vi "SetReadTrigger.vi"() -> ()   [LabVIEW 2015]
panel:
  out "触发状态":string
  in  "VISA资源名称":refnum<visa-resource-name>
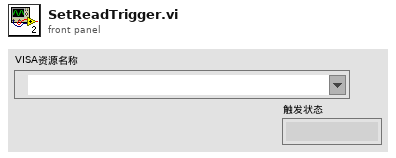
[diagram p1: front panel]
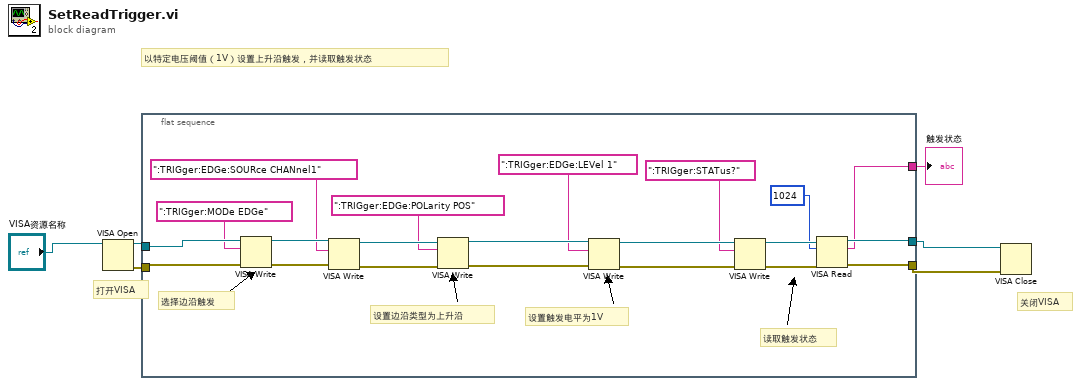
[diagram p0: block diagram]
diagram:
  # "关闭VISA"
  # "打开VISA"
  # "以特定电压阈值（1V）设置上升沿触发，并读取触发状态"
  n1 = VISA Open(VISA resource name="VISA资源名称") -> (VISA resource name=w6:refnum<visa-resource-name>, error out=w5:errorcluster)  [unwired: 4 in]
  n2 = flat-sequence {
    tunnel: w6 -> [w27]
    tunnel: w5 -> [w26]
    tunnel: [w11] -> w3
    tunnel: [w9] -> w2
    tunnel: [w7] -> w1
    frame #0 {
      # "设置触发电平为1V"
      # "设置边沿类型为上升沿"
      # "读取触发状态"
      # "选择边沿触发"
      n3 = VISA Write(VISA resource name=w27, write buffer=":TRIGger:MODe EDGe", error in (no error)=w26) -> (VISA resource name out=w24:refnum<visa-resource-name>, error out=w22:errorcluster)  [unwired: 1 out]
      n4 = VISA Write(VISA resource name=w24, write buffer=":TRIGger:EDGe:SOURce CHANnel1" ("写入缓冲区"), error in (no error)=w22) -> (VISA resource name out=w23:refnum<visa-resource-name>, error out=w21:errorcluster)  [unwired: 1 out]
      n5 = VISA Write(VISA resource name=w23, write buffer=":TRIGger:EDGe:POLarity POS" ("写入缓冲区"), error in (no error)=w21) -> (VISA resource name out=w18:refnum<visa-resource-name>, error out=w17:errorcluster)  [unwired: 1 out]
      n6 = VISA Write(VISA resource name=w18, write buffer=":TRIGger:EDGe:LEVel 1" ("写入缓冲区"), error in (no error)=w17) -> (VISA resource name out=w15:refnum<visa-resource-name>, error out=w14:errorcluster)  [unwired: 1 out]
      n7 = VISA Write(VISA resource name=w15, write buffer=":TRIGger:STATus?" ("写入缓冲区"), error in (no error)=w14) -> (VISA resource name out=w12:refnum<visa-resource-name>, error out=w10:errorcluster)  [unwired: 1 out]
      n8 = VISA Read(VISA resource name=w12, byte count=u32 1024 ("字节总数"), error in (no error)=w10) -> (VISA resource name out=w11:refnum<visa-resource-name>, read buffer=w7:string, error out=w9:errorcluster)  [unwired: 1 out]
    }
  }
  n9 = VISA Close(VISA resource name=w3, error in (no error)=w2) -> ()  [unwired: 1 out]
  "触发状态" <- w1
